vi "Get CAN Status.vi"(6 "timeout (ms)":i32=5000, 8 "error in":errorcluster, 11 "gRPC ID":T4) -> (0 "error out":errorcluster, 2 "CAN Status":T1, 3 "gRPC ID out":T4)   [LabVIEW 2021, in "CAN_Writer_NIXNET_Wrapper.lvlib"]
uses:
  <vilib>/gRPC/LabVIEW gRPC Library/Shared/grpcId.ctl
  CAN_Writer_NIXNET_Wrapper.lvlib
  CanWriterNixnet_client/CanWriterNixnet_client.lvlib
  <vilib>/CIF Foundation/CIF CAN RW Core/typedef/Communication State.ctl
  <vilib>/CIF Foundation/CIF CAN RW Core/CAN_RW_CORE.lvclass
  <vilib>/CIF Foundation/CIF CAN RW Core/typedef/Last Error.ctl
  <vilib>/CIF Foundation/CIF CAN RW Core/typedef/CAN Status.ctl
  <vilib>/gRPC/LabVIEW gRPC Library/grpc-lvsupport-release.lvlib
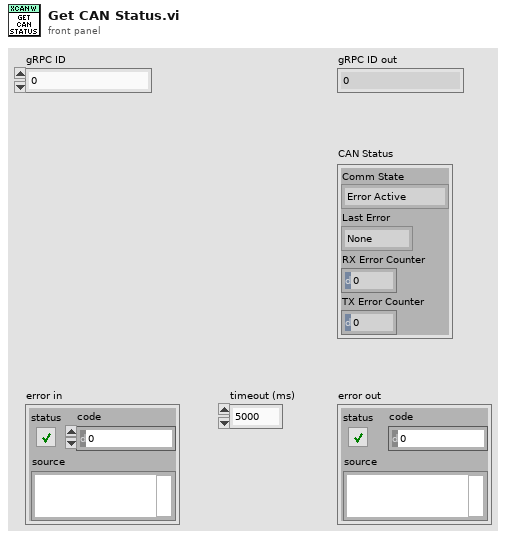
[diagram p1: front panel]
types:
  T1 = typedef "CAN_RW_CORE.lvclass/CAN Status.ctl" = cluster{"Comm State":T2, "Last Error":T3, "RX Error Counter":u8, "TX Error Counter":u8}
  T2 = typedef "CAN_RW_CORE.lvclass/Communication State.ctl" = enum16{"Error Active", "Error Passive", "Bus Off"}
  T3 = typedef "CAN_RW_CORE.lvclass/Last Error.ctl" = enum16{"None", "Stuff", "Form", "Ack", "Bit1", "Bit0", "CRC", "Unknown"}
  T4 = typedef "grpc-lvsupport-release.lvlib/grpcId.ctl" = u64
  T5 = typedef "CanWriterNixnet_client.lvlib/cif_can_writer_nixnet_GetCANStatusResponse.ctl" = cluster{"comm_state":T6, "last_error":T7, "rx_error_ctr":u32, "tx_error_crt":u32}
  T6 = typedef "CanWriterNixnet_client.lvlib/cif_can_writer_nixnet_CommState.ctl" = enum32{"COMMSTATE_ERROR_ACTIVE", "COMMSTATE_ERROR_PASSIVE", "COMMSTATE_BUS_OFF"}
  T7 = typedef "CanWriterNixnet_client.lvlib/cif_can_writer_nixnet_LastError.ctl" = enum32{"LASTERROR_NONE", "LASTERROR_STUFF", "LASTERROR_FORM", "LASTERROR_ACK", "LASTERROR_BIT1", "LASTERROR_BIT0", "LASTERROR_CRC", "LASTERROR_UNKNOWN"}
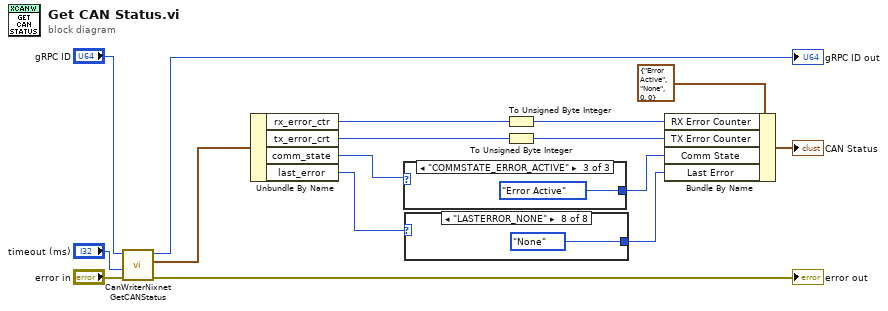
[diagram p0: block diagram]
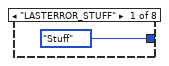
[diagram p2: hidden frame]
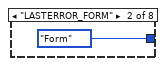
[diagram p3: hidden frame]
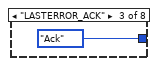
[diagram p4: hidden frame]
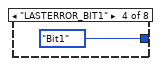
[diagram p5: hidden frame]
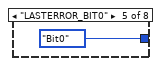
[diagram p6: hidden frame]
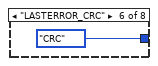
[diagram p7: hidden frame]
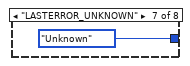
[diagram p8: hidden frame]
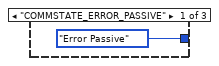
[diagram p9: hidden frame]
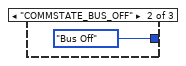
[diagram p10: hidden frame]
diagram:
  n1 = call "CanWriterNixnet GetCANStatus.vi"("error in"="error in", "timeout (ms)"="timeout (ms)", "gRPC ID"="gRPC ID") -> ("error out"=→"error out":errorcluster, "Response Data"=w11:T5, "gRPC ID out"=→"gRPC ID out":T4)  [unwired: 6 in]
  n2 = Unbundle By Name(w11) -> ("rx_error_ctr"=w9:u32, "tx_error_crt"=w7:u32, "comm_state"=w5:T6, "last_error"=w3:T7)
  n3 = case shown="\"COMMSTATE_ERROR_ACTIVE\"" w5 {
    tunnel: [Communication_State."Error Passive" ("Comm State") Communication_State."Bus Off" ("Comm State") Communication_State."Error Active" ("Comm State")] -> w4
    frame "COMMSTATE_ERROR_PASSIVE" {
    }
    frame "COMMSTATE_BUS_OFF" {
    }
    frame "COMMSTATE_ERROR_ACTIVE" {
    }
  }
  n4 = case shown="\"LASTERROR_NONE\"" w3 {
    tunnel: [Last_Error."Stuff" ("Last Error") Last_Error."Form" ("Last Error") Last_Error."Ack" ("Last Error") Last_Error."Bit1" ("Last Error") Last_Error."Bit0" ("Last Error") Last_Error."CRC" ("Last Error") Last_Error."Unknown" ("Last Error") Last_Error."None" ("Last Error")] -> w2
    frame "LASTERROR_STUFF" {
    }
    frame "LASTERROR_FORM" {
    }
    frame "LASTERROR_ACK" {
    }
    frame "LASTERROR_BIT1" {
    }
    frame "LASTERROR_BIT0" {
    }
    frame "LASTERROR_CRC" {
    }
    frame "LASTERROR_UNKNOWN" {
    }
    frame "LASTERROR_NONE" {
    }
  }
  n5 = To Unsigned Byte Integer(number=w9) -> (unsigned 8bit integer=w8:u8)
  n6 = To Unsigned Byte Integer(number=w7) -> (unsigned 8bit integer=w6:u8)
  n7 = Bundle By Name(cluster=T1 {"Comm State"=enum."Error Active", "Last Error"=enum."None", "RX Error Counter"=0, "TX Error Counter"=0} ("CAN Status"), "RX Error Counter"=w8, "TX Error Counter"=w6, "Comm State"=w4, "Last Error"=w2) -> (→"CAN Status":T1)
